vi "Upgrade Addon to Latest Version.vi"(8 "error in (no error)":errorcluster, 11 "Device Item Ref in in":T1 format="%.0x") -> (0 "error out":errorcluster, 3 "Device Item Ref out":T1 format="%.0x")   [LabVIEW 2019, in "Control Addon Shared.lvlib"]
uses:
  Control Addon Shared.lvlib
  <vilib>/NI VeriStand/Custom Device API/Custom Device Item Ref.ctl
  NationalInstruments.VeriStand.SystemDefinitionAPI
  Constants.vi
  <vilib>/NI/NI VeriStand Advanced SysDef API/SysDef API/Advanced System Definition.lvlib
  <vilib>/NI VeriStand/Custom Device API/Custom Device API.lvlib
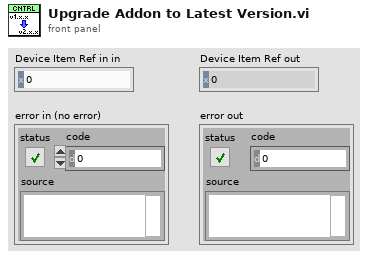
[diagram p1: front panel]
types:
  T1 = typedef "Custom Device API.lvlib/Custom Device Item Ref.ctl" = u64
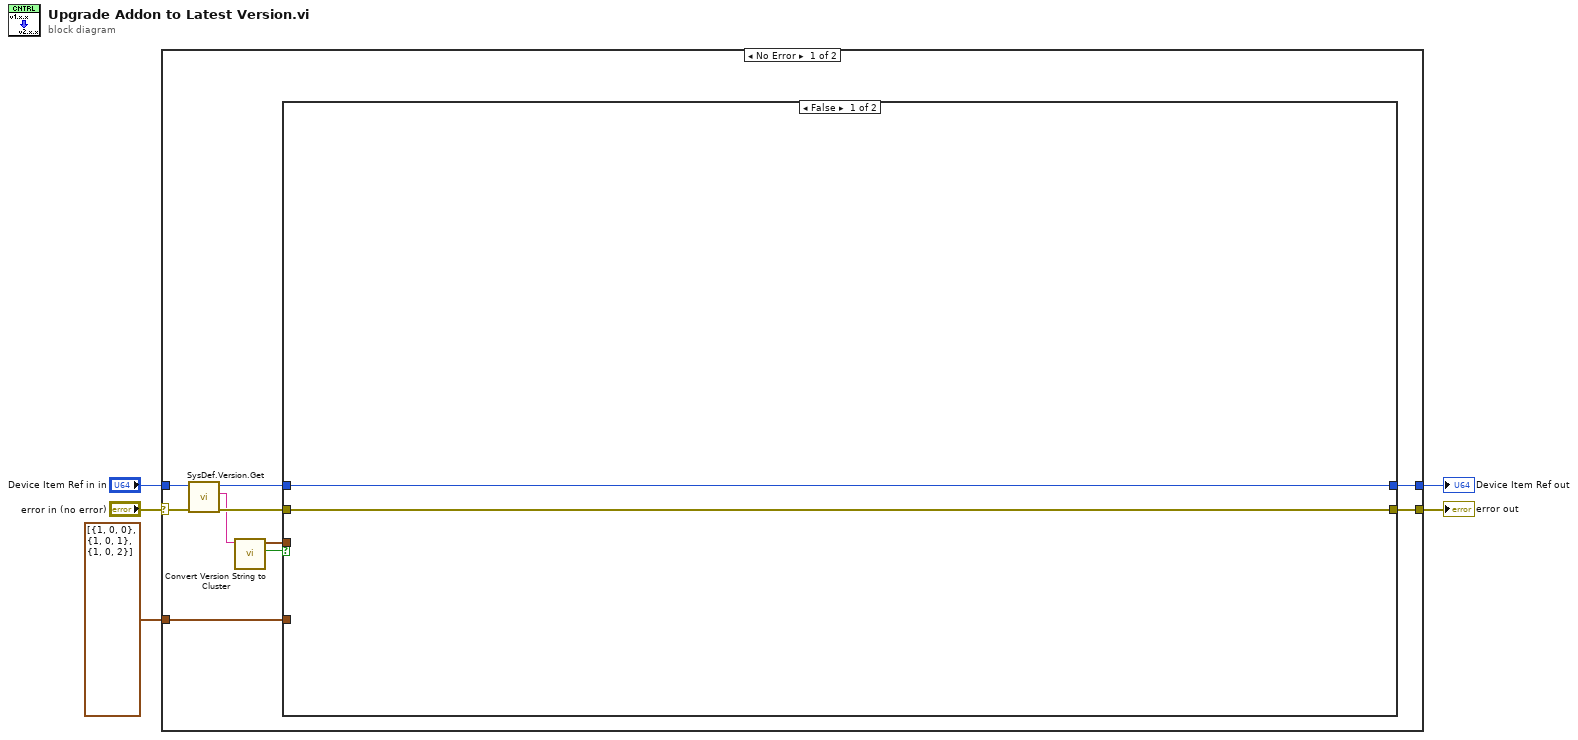
[diagram p0: block diagram]
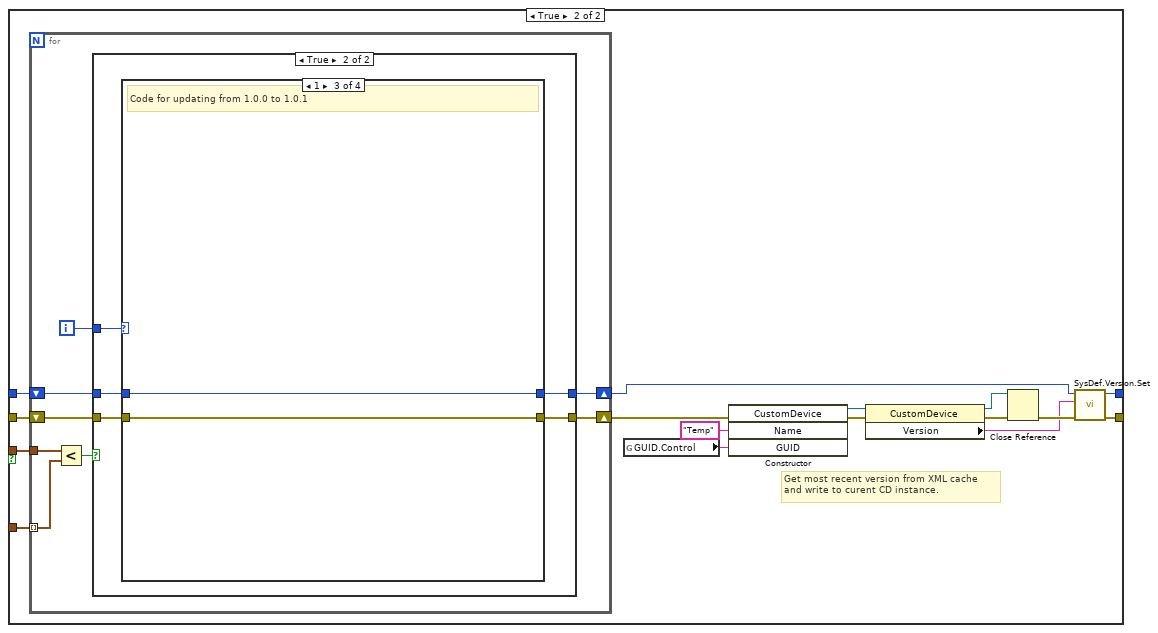
[diagram p2: hidden frame]
diagram:
  n1 = case shown="No Error" "error in (no error)" {
    selector: "error in (no error)" -> [w12 w58]
    tunnel: [w14 w58] -> w4
    tunnel: "Device Item Ref in in" -> [w11 w57]
    tunnel: [w13 w57] -> w5
    tunnel: cluster{i32, i32, i32}[] [{1, 0, 0}, {1, 0, 1}, {1, 0, 2}] -> [w15 _]
    frame No Error {
      n2 = call <vilib>:"SysDef.Version.Get.vi"("error in (no error)"=w12, "nodeID"=w11) -> ("error out"=w10:errorcluster, "Version"=w8:string, "nodeID out"=w9:u64)  [unwired: 7 in]
      n3 = call "Convert Version String to Cluster.vi"("Version"=w8) -> ("Version Valid?"=w6:bool, "Version"=w7:cluster{i32, i32, i32})  [unwired: 9 in]
      n4 = case shown="False" w6 {
        tunnel: w15 -> [_ w33]
        tunnel: [w16 w26] -> w14
        tunnel: [w17 w25] -> w13
        tunnel: w10 -> [w16 w21]
        tunnel: w9 -> [w17 w20]
        tunnel: w7 -> [_ w18]
        frame False {
        }
        frame True {
          # "Get most recent version from XML cache\nand write to curent CD instance."
          n5 = for {
            tunnel: w33 -> [w39] mode=indexing
            shift-right: [w41] -> w24
            shift-left: w21 -> [w35]
            shift-right: [w40] -> w23
            shift-left: w20 -> [w34]
            tunnel: w18 -> [w36]
            i -> [w37]
            n6 = Less?(x=w36, y=w39) -> (x < y?=w38:bool)
            n7 = case shown="True" w38 {
              tunnel: w35 -> [w43 w48]
              tunnel: [w43 w47] -> w41
              tunnel: w34 -> [w42 w44]
              tunnel: [w42 w45] -> w40
              tunnel: w37 -> [_ w46]
              frame False {
              }
              frame True {
                n8 = case shown="1" w46 {
                  tunnel: w48 -> [w50 w52 w54 w56]
                  tunnel: [w50 w52 w54 w56] -> w47
                  tunnel: [w49 w51 w53 w55] -> w45
                  tunnel: w44 -> [w49 w51 w53 w55]
                  frame Default {
                    # "Nothing to update"
                  }
                  frame 0 {
                    # "Initial Onload"
                  }
                  frame 1 {
                    # "Code for updating from 1.0.0 to 1.0.1"
                  }
                  frame 2 {
                    # "Code for updating from 1.0.1 to 1.0.2"
                  }
                }
              }
            }
          }
          n9 = global read "Constants.vi" "GUID.Control"() -> (w19:string)
          n10 = constructor class="CustomDevice"(error in=w24, "Name"="Temp", "GUID"=w19) -> (reference out=w32:refnum<k24>, error out=w31:errorcluster)  [unwired: 2 in, 3 out]
          n11 = property class="CustomDevice"(reference=w32, error in=w31) -> (reference out=w29:refnum<k24>, error out=w30:errorcluster, "Version"=w27:string)
          n12 = Close Reference(reference=w29, error in (no error)=w30) -> (error out=w28:errorcluster)
          n13 = call <vilib>:"SysDef.Version.Set.vi"("error in (no error)"=w28, "Version"=w27, "nodeID"=w23) -> ("error out"=w26:errorcluster, "nodeID out"=w25:u64)  [unwired: 7 in]
        }
      }
    }
    frame Error {
    }
  }
  "Device Item Ref out" <- w5
  "error out" <- w4
